vi "Condition_Evaluate.vi"(8 "error in (no error)":errorcluster={"status"=FALSE, "code"=0, "source"="\"\""}, 9 "tolerance":dbl=2.0, 10 "target_setpoint":dbl=100.0, 11 "actual_value":dbl=100.0) -> (0 "error out":errorcluster={"status"=FALSE, "code"=0, "source"="\"\""}, 3 "condition_met":bool)   [LabVIEW 2026]
doc: "INTENT: Evaluate parameter value against setpoint target and tolerance."
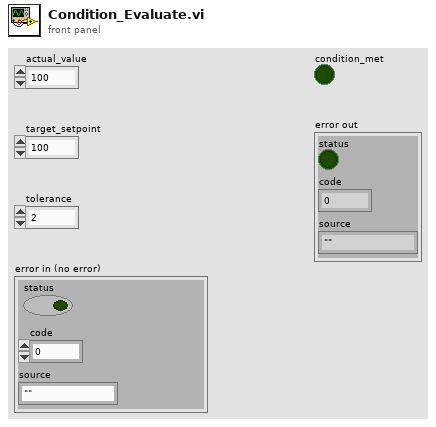
[diagram p1: front panel]
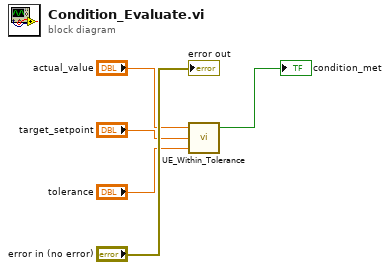
[diagram p0: block diagram]
diagram:
  n1 = call "UE_Within_Tolerance.vi"("tolerance"="tolerance", "target"="target_setpoint", "actual"="actual_value") -> ("within_tolerance"=→"condition_met":bool)  [unwired: 2 in]
  "error out" <- "error in (no error)"
